vi "MakeMeasurement.vi"(8 "references":T1, 11 "measurement setting":T2) -> (0 "references out":T1, 3 "measurement":T3)   [LabVIEW 2011]
doc: "Performs one measurement for the given measurement settings, reads out Sources values and temperature of voltmeter."
uses:
  Measurement Setting.ctl
  Measurement References.ctl
  <vilib>/Utility/NIReport.llb/NI_report.lvclass
  <instrlib>/Fluke 5XXX Series Multicalibrators/Fluke 5XXX Series Multicalibrators.lvlib
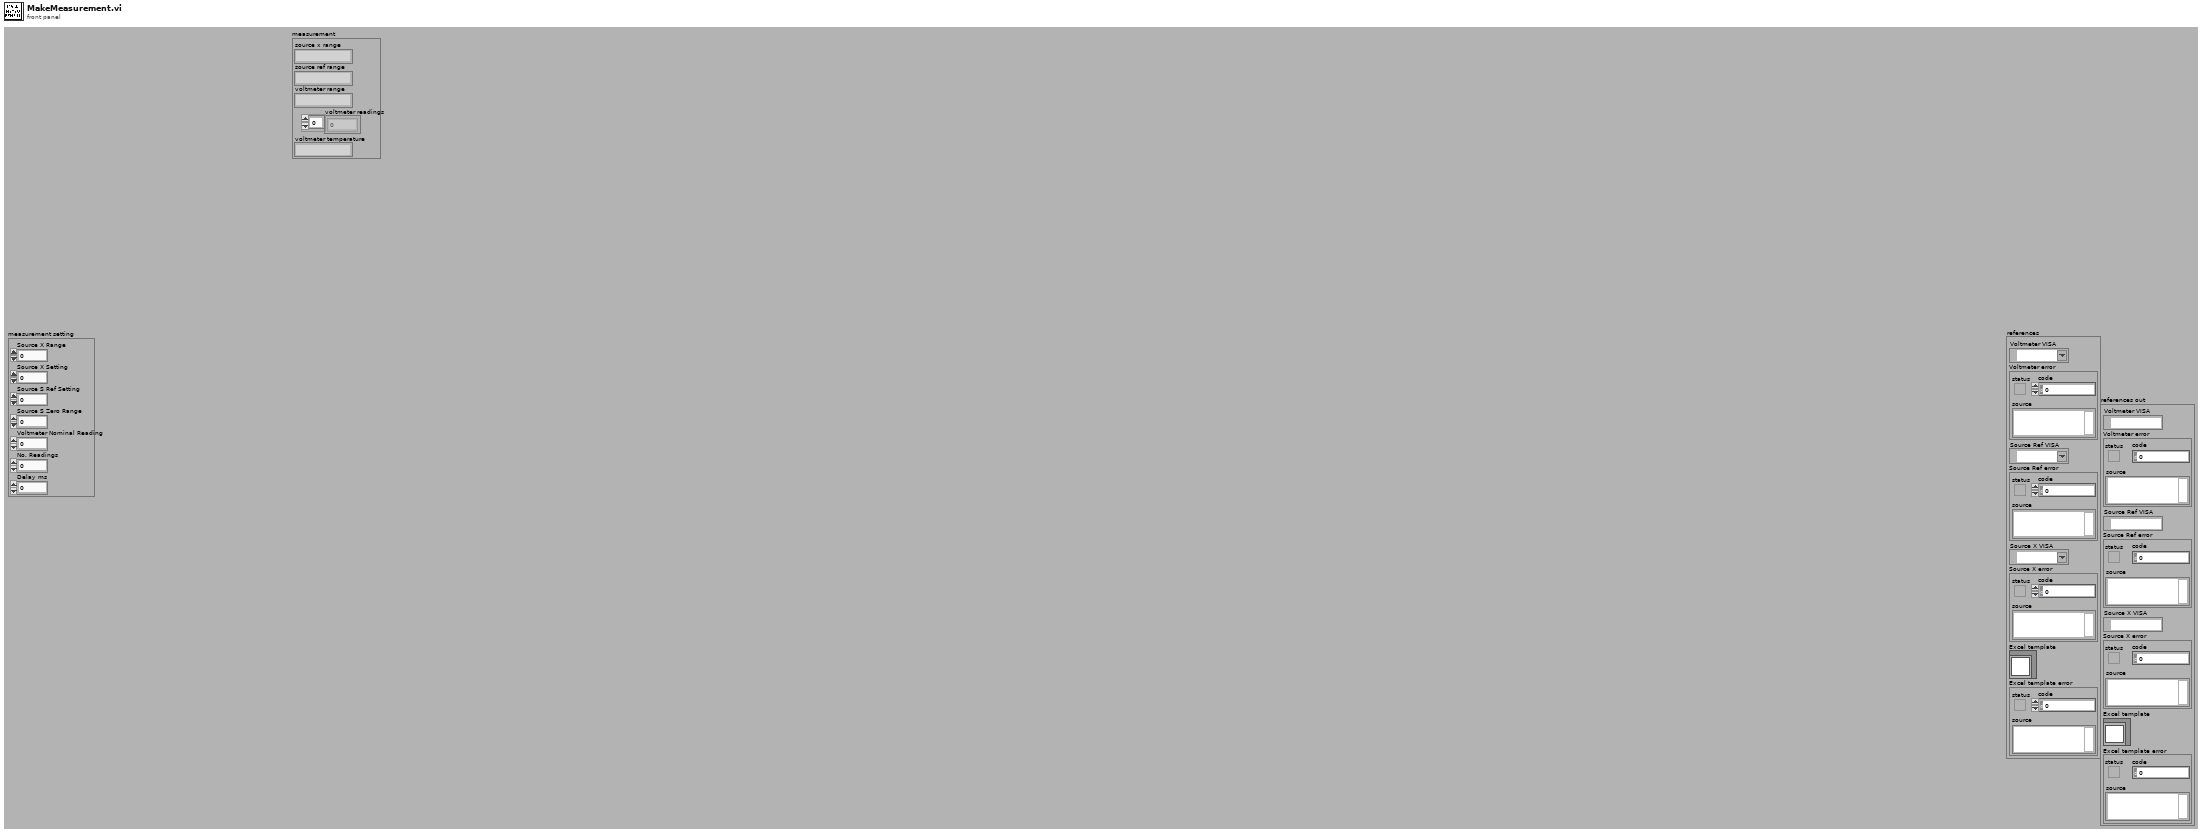
[diagram p1: front panel]
types:
  T1 = typedef "Measurement References.ctl" = cluster{"Voltmeter VISA":refnum<visa-resource-name>, "Voltmeter error":errorcluster, "Source Ref VISA":refnum<visa-resource-name>, "Source Ref error":errorcluster, "Source X VISA":refnum<visa-resource-name>, "Source X error":errorcluster, "Excel template":refnum<class "NI_report.lvclass">, "Excel template error":errorcluster}
  T2 = typedef "Measurement Setting.ctl" = cluster{"Source X Range":dbl, "Source X Setting":dbl, "Source S Ref Setting":dbl, "Source S Zero Range":dbl, "Voltmeter Nominal Reading":dbl, "No. Readings":dbl, "Delay ms":dbl}
  T3 = cluster{"source x range":string, "source ref range":string, "voltmeter range":string, "voltmeter readings":dbl[], "voltmeter temperature":string}
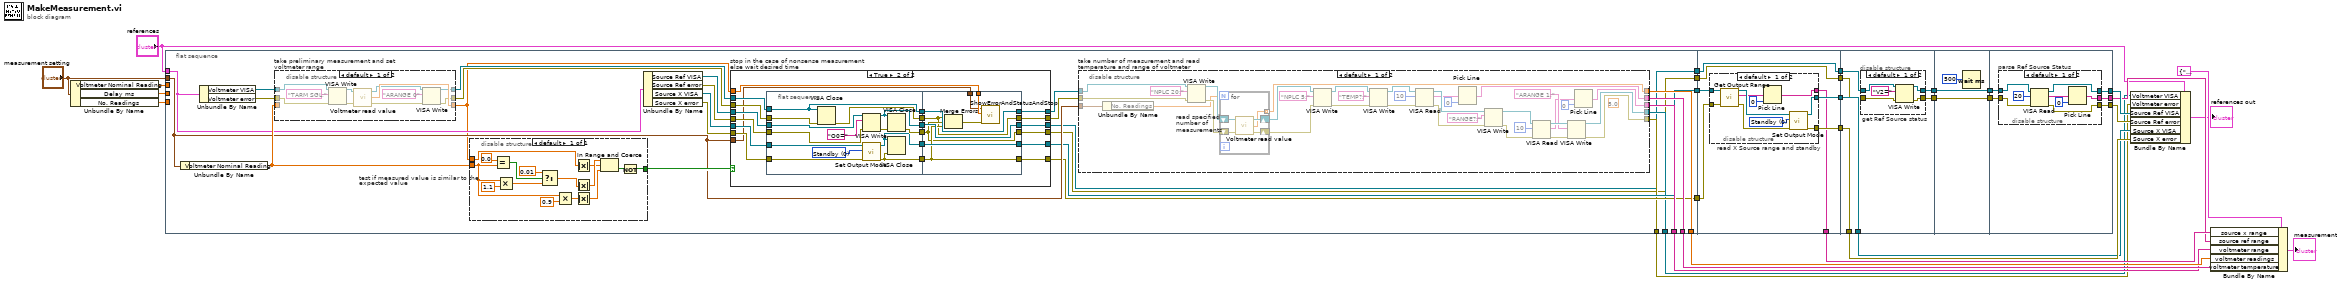
[diagram p0: block diagram]
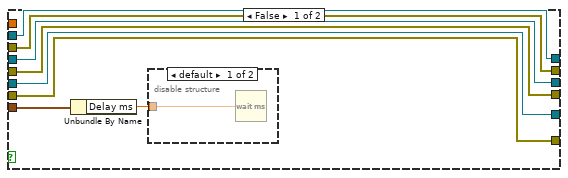
[diagram p2: hidden frame]
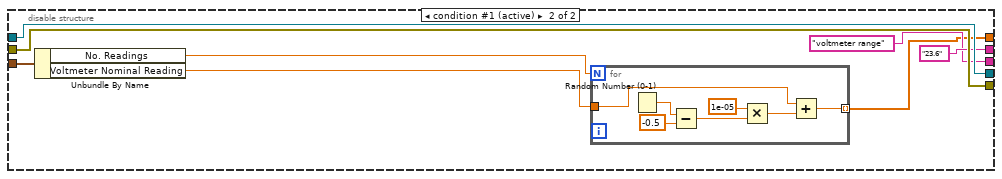
[diagram p4: hidden frame]
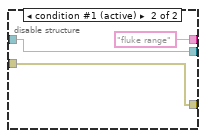
[diagram p6: hidden frame]
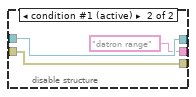
[diagram p8: hidden frame]
diagram:
  n1 = Unbundle By Name("measurement setting") -> ("Voltmeter Nominal Reading"=w6:dbl, "Delay ms"=w5:dbl, "No. Readings"=w4:dbl)
  n2 = flat-sequence {
    tunnel: w6 -> [_]
    tunnel: w5 -> [_]
    tunnel: w4 -> [_]
    tunnel: [w55] -> w25
    tunnel: [w54] -> w19
    tunnel: [w53] -> w16
    tunnel: "measurement setting" -> [w46]
    tunnel: [w45] -> w14
    tunnel: [w44] -> w13
    tunnel: [w43] -> w12
    tunnel: [w42] -> w11
    tunnel: "references" -> [w37]
    tunnel: [w36] -> w9
    tunnel: [w35] -> w8
    tunnel: [w197] -> w31
    tunnel: [w196] -> w30
    tunnel: [w195] -> w18
    tunnel: w14 -> [w194]
    tunnel: w13 -> [w193]
    tunnel: [w192] -> w10
    tunnel: w9 -> [w192]
    tunnel: w8 -> [w191]
    tunnel: [w191] -> w7
    tunnel: [w216] -> w29
    tunnel: [w215] -> w28
    tunnel: w31 -> [w214]
    tunnel: w30 -> [w213]
    tunnel: [w213] -> w23
    tunnel: [w214] -> w22
    tunnel: w10 -> [w212]
    tunnel: w7 -> [w211]
    tunnel: [w225] -> w27
    tunnel: w29 -> [w225]
    tunnel: w28 -> [w224]
    tunnel: [w224] -> w26
    tunnel: w27 -> [w231]
    tunnel: w26 -> [w230]
    tunnel: [w229] -> w20
    tunnel: [w228] -> w21
    tunnel: [w227] -> w17
    frame #0 {
      n3 = Unbundle By Name(w46) -> ("Voltmeter Nominal Reading"=w47:dbl)
      n4 = Unbundle By Name(w37) -> ("Voltmeter VISA"=w33:refnum<visa-resource-name>, "Voltmeter error"=w32:errorcluster)
      n5 = disable-structure "take preliminary measurement and set voltmeter range" shown="default" {
        disable-tunnel: w33 -> [w183 w189]
        disable-tunnel: w32 -> [w186 w190]
        disable-tunnel: [w187 w188] -> w34
        disable-tunnel: [w180 w190] -> w49
        disable-tunnel: [w178 w189] -> w51
        disable-tunnel: w47 -> [_ w188]
        frame condition #0 {
          n6 = VISA Write(VISA resource name=w183, write buffer="TARM SGL;", error in (no error)=w186) -> (VISA resource name out=w184:refnum<visa-resource-name>, error out=w185:errorcluster)  [unwired: 1 out]
          n7 = call "Voltmeter read value.vi"("error in"=w185, "Voltmeter VISA in"=w184) -> ("error out"=w181:errorcluster, "Value"=w187:dbl, "Voltmeter VISA"=w179:refnum<visa-resource-name>)  [unwired: 1 in]
          n8 = VISA Write(VISA resource name=w179, write buffer="ARANGE 0", error in (no error)=w181) -> (VISA resource name out=w178:refnum<visa-resource-name>, error out=w180:errorcluster)  [unwired: 1 out]
        }
        frame condition #1 (active) {
        }
      }
      n9 = disable-structure "test if measured value is similar to the expected value" shown="default" {
        disable-tunnel: w34 -> [w64]
        disable-tunnel: w47 -> [w62]
        disable-tunnel: [w56] -> w52
        frame Enabled {
          n10 = Equal?(x=0.0 ("y"), y=w62) -> (x = y?=w60:bool)
          n11 = Multiply(x=w62, y=1.1) -> (x*y=w59:dbl)
          n12 = Select(t=0.01, s=w60, f=w59) -> (s? t:f=w57:dbl)
          n13 = Multiply(x=w62, y=0.9) -> (x*y=w67:dbl)
          n14 = Absolute Value(x=w64) -> (abs(x)=w65:dbl)
          n15 = Absolute Value(x=w57) -> (abs(x)=w68:dbl)
          n16 = Absolute Value(x=w67) -> (abs(x)=w66:dbl)
          n17 = In Range and Coerce(upper limit=w68, x=w65, lower limit=w66) -> (In Range?=w63:bool)  [unwired: 1 out]
          n18 = Not(x=w63) -> (.not. x?=w56:bool)
        }
      }
      n19 = Unbundle By Name(w37) -> ("Source Ref VISA"=w38:refnum<visa-resource-name>, "Source Ref error"=w39:errorcluster, "Source X VISA"=w40:refnum<visa-resource-name>, "Source X error"=w41:errorcluster)
      n20 = case "stop in the case of nonsense measurement else wait desired time" shown="True" w52 {
        tunnel: w38 -> [w78 w97]
        tunnel: w39 -> [w77 w96]
        tunnel: w40 -> [w76 w99]
        tunnel: w41 -> [w75 w98]
        tunnel: [w78 w95] -> w36
        tunnel: [w77 w94] -> w35
        tunnel: [w76 w92] -> w45
        tunnel: [w75 w93] -> w44
        tunnel: w51 -> [w74 w91]
        tunnel: [w74 w88] -> w50
        tunnel: w49 -> [w73 w90]
        tunnel: [w73 w89] -> w48
        tunnel: w46 -> [w72 w80]
        tunnel: w34 -> [_ w81]
        frame False {
          n21 = Unbundle By Name(w72) -> ("Delay ms"=w71:dbl)
          n22 = disable-structure shown="default" {
            disable-tunnel: w71 -> [w79 _]
            frame condition #0 {
              n23 = Wait (ms)(milliseconds to wait=w79) -> ()  [unwired: 1 out]
            }
            frame condition #1 (active) {
            }
          }
        }
        frame True {
          n24 = flat-sequence {
            tunnel: w99 -> [w113]
            tunnel: w98 -> [w112]
            tunnel: w97 -> [w109]
            tunnel: w96 -> [w108]
            tunnel: w91 -> [w100]
            tunnel: w90 -> [w102]
            tunnel: [w107] -> w87
            tunnel: [w105] -> w86
            tunnel: [w104] -> w85
            tunnel: [w103] -> w84
            tunnel: [w101] -> w83
            tunnel: [w100] -> w82
            tunnel: [w121] -> w92
            tunnel: [w119] -> w93
            tunnel: [w118] -> w94
            tunnel: [w122] -> w95
            tunnel: [w117] -> w89
            tunnel: [w120] -> w88
            tunnel: w80 -> [w114]
            tunnel: w81 -> [w115]
            tunnel: w82 -> [w120]
            tunnel: w83 -> [w117]
            tunnel: w84 -> [w121]
            tunnel: w85 -> [w119]
            tunnel: w86 -> [w118]
            tunnel: w87 -> [w122]
            frame #0 {
              w111 = u32 0 items=["Standby", "Operate"] ("Output Mode (0: Standby)")
              n25 = VISA Close(VISA resource name=w100, error in (no error)=w102) -> (error out=w101:errorcluster)
              n26 = VISA Write(VISA resource name=w109, write buffer="O0=", error in (no error)=w108) -> (VISA resource name out=w107:refnum<visa-resource-name>, error out=w106:errorcluster)  [unwired: 1 out]
              n27 = call <instrlib>:"Set Output Mode.vi"("error in (no error)"=w112, "Output Mode (0: Standby)"=w111, "VISA resource name"=w113) -> ("error out"=w104:errorcluster, "VISA resource name out"=w103:refnum<visa-resource-name>)  [unwired: 7 in]
              n28 = VISA Close(VISA resource name=w107, error in (no error)=w106) -> (error out=w105:errorcluster)
              n29 = VISA Close(VISA resource name=w103, error in (no error)=w104) -> ()  [unwired: 1 out]
            }
            frame #1 {
              n30 = Merge Errors(w117, w118, w119) -> (w116:errorcluster)
              n31 = call "ShowErrorAndStatusAndStop.vi"("error in"=w116, "measured value in"=w115, "measurement setting in"=w114) -> ()  [unwired: 9 in]
            }
          }
        }
      }
      n32 = disable-structure "take number of measurement and read temperature and range of voltmeter" shown="default" {
        disable-tunnel: w48 -> [w150 w168]
        disable-tunnel: w50 -> [w149 w169]
        disable-tunnel: [w144 w165] -> w55
        disable-tunnel: [w130 "23.6" ("read buffer")] -> w54
        disable-tunnel: [w138 w169] -> w43
        disable-tunnel: [w137 w168] -> w42
        disable-tunnel: [w123 "voltmeter range" ("read buffer")] -> w53
        disable-tunnel: w46 -> [w146 w162]
        frame condition #0 {
          (unwired) 5.0 ("Integration Time (0 PLCs)")
          n33 = Unbundle By Name(w146) -> ("No. Readings"=w136:dbl)
          n34 = VISA Write(VISA resource name=w149, write buffer="NPLC 20;", error in (no error)=w150) -> (VISA resource name out=w148:refnum<visa-resource-name>, error out=w147:errorcluster)  [unwired: 1 out]
          n35 = for "read specified\nnumber of\nmeasurements" {
            N: w136 -> [_]
            shift-right: [w158] -> w143
            shift-left: w147 -> [w159]
            shift-right: [w160] -> w141
            shift-left: w148 -> [w161]
            tunnel: [w157] -> w144 mode=indexing
            n36 = call "Voltmeter read value.vi"("error in"=w159, "Voltmeter VISA in"=w161) -> ("error out"=w158:errorcluster, "Value"=w157:dbl, "Voltmeter VISA"=w160:refnum<visa-resource-name>)  [unwired: 1 in]
          }
          n37 = VISA Write(VISA resource name=w141, write buffer="NPLC 5;", error in (no error)=w143) -> (VISA resource name out=w140:refnum<visa-resource-name>, error out=w142:errorcluster)  [unwired: 1 out]
          n38 = VISA Write(VISA resource name=w140, write buffer="TEMP?;", error in (no error)=w142) -> (VISA resource name out=w154:refnum<visa-resource-name>, error out=w155:errorcluster)  [unwired: 1 out]
          n39 = VISA Read(VISA resource name=w154, byte count=u32 10, error in (no error)=w155) -> (VISA resource name out=w152:refnum<visa-resource-name>, read buffer=w132:string, error out=w151:errorcluster)  [unwired: 1 out]
          n40 = Pick Line(multi-line string=w132, line index=0) -> (output string=w130:string)  [unwired: 1 in]
          n41 = VISA Write(VISA resource name=w152, write buffer="RANGE?;", error in (no error)=w151) -> (VISA resource name out=w128:refnum<visa-resource-name>, error out=w129:errorcluster)  [unwired: 1 out]
          n42 = VISA Read(VISA resource name=w128, byte count=u32 10, error in (no error)=w129) -> (VISA resource name out=w134:refnum<visa-resource-name>, read buffer=w124:string, error out=w135:errorcluster)  [unwired: 1 out]
          n43 = VISA Write(VISA resource name=w134, write buffer="ARANGE 1;", error in (no error)=w135) -> (VISA resource name out=w138:refnum<visa-resource-name>, error out=w137:errorcluster)  [unwired: 1 out]
          n44 = Pick Line(multi-line string=w124, line index=0) -> (output string=w123:string)  [unwired: 1 in]
        }
        frame condition #1 (active) {
          n45 = Unbundle By Name(w162) -> ("No. Readings"=w164:dbl, "Voltmeter Nominal Reading"=w163:dbl)
          n46 = for {
            N: w164 -> [_]
            tunnel: w163 -> [w176]
            tunnel: [w170] -> w165 mode=indexing
            n47 = Random Number (0-1)() -> (number: 0 to 1=w175:dbl)
            n48 = Subtract(x=w175, y=-0.5) -> (x-y=w173:dbl)
            n49 = Multiply(x=1e-05, y=w173) -> (x*y=w171:dbl)
            n50 = Add(x=w176, y=w171) -> (x+y=w170:dbl)
          }
        }
      }
    }
    frame #1 {
      n51 = disable-structure "read X Source range and standby" shown="default" {
        disable-tunnel: w194 -> [w207 w210]
        disable-tunnel: w193 -> [w206 w209]
        disable-tunnel: [w202 w210] -> w197
        disable-tunnel: [w201 w209] -> w196
        disable-tunnel: [w198 "fluke range" ("Primary Output")] -> w195
        frame condition #0 {
          w203 = u32 0 items=["Standby", "Operate"] ("Output Mode (0: Standby)")
          n52 = call <instrlib>:"Get Output Range.vi"("error in (no error)"=w206, "VISA resource name"=w207) -> ("error out"=w204:errorcluster, "Primary Output"=w200:string, "VISA resource name out"=w205:refnum<visa-resource-name>)  [unwired: 6 in, 1 out]
          n53 = Pick Line(multi-line string=w200, line index=0) -> (output string=w198:string)  [unwired: 1 in]
          n54 = call <instrlib>:"Set Output Mode.vi"("error in (no error)"=w204, "Output Mode (0: Standby)"=w203, "VISA resource name"=w205) -> ("error out"=w201:errorcluster, "VISA resource name out"=w202:refnum<visa-resource-name>)  [unwired: 7 in]
        }
        frame condition #1 (active) {
        }
      }
    }
    frame #2 {
      n55 = disable-structure "get Ref Source status" shown="default" {
        disable-tunnel: w212 -> [w221 w223]
        disable-tunnel: w211 -> [w220 w222]
        disable-tunnel: [w218 w223] -> w216
        disable-tunnel: [w217 w222] -> w215
        frame condition #0 {
          n56 = VISA Write(VISA resource name=w221, write buffer="V2=", error in (no error)=w220) -> (VISA resource name out=w218:refnum<visa-resource-name>, error out=w217:errorcluster)  [unwired: 1 out]
        }
        frame condition #1 (active) {
        }
      }
    }
    frame #3 {
      n57 = Wait (ms)(milliseconds to wait=u32 500) -> ()  [unwired: 1 out]
    }
    frame #4 {
      n58 = disable-structure "parse Ref Source Status" shown="default" {
        disable-tunnel: w231 -> [w239 w242]
        disable-tunnel: w230 -> [w238 w241]
        disable-tunnel: [w236 w242] -> w229
        disable-tunnel: [w235 w241] -> w228
        disable-tunnel: [w232 "datron range" ("read buffer")] -> w227
        frame condition #0 {
          n59 = VISA Read(VISA resource name=w239, byte count=u32 20, error in (no error)=w238) -> (VISA resource name out=w236:refnum<visa-resource-name>, read buffer=w234:string, error out=w235:errorcluster)  [unwired: 1 out]
          n60 = Pick Line(multi-line string=w234, line index=0) -> (output string=w232:string)  [unwired: 1 in]
        }
        frame condition #1 (active) {
        }
      }
    }
  }
  n61 = Bundle By Name(cluster="references", "Voltmeter VISA"=w12, "Voltmeter error"=w11, "Source Ref VISA"=w20, "Source Ref error"=w21, "Source X VISA"=w22, "Source X error"=w23) -> (→"references out":T1)
  n62 = Bundle By Name(cluster=T3 {"source x range"="", "source ref range"="", "voltmeter range"="", "voltmeter readings"=[], "voltmeter temperature"=""}, "source x range"=w18, "source ref range"=w17, "voltmeter range"=w16, "voltmeter readings"=w25, "voltmeter temperature"=w19) -> (→"measurement":T3)
